vi "Scaled Value.vi"(8 "error in":errorcluster, 11 "Sensor in":refnum<class "Sensor.lvclass">) -> (0 "error out":errorcluster, 2 "Scaled Value":dbl, 3 "Sensor out":refnum<class "Sensor.lvclass">)   [LabVIEW 2026, in "Sensor.lvclass"]
doc: "Returns the sensor's Value multiplied by its Gain. Both fields are read through the class's own Read accessors; the object passes through unchanged."
uses:
  Sensor.lvclass
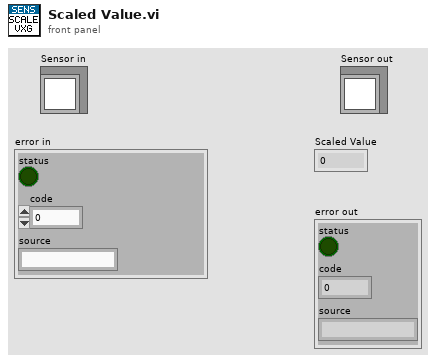
[diagram p1: front panel]
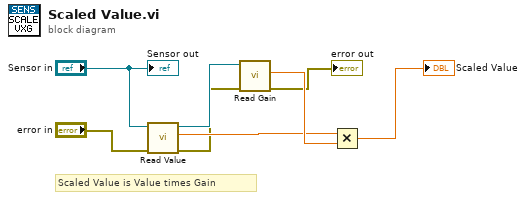
[diagram p0: block diagram]
diagram:
  # "Scaled Value is Value times Gain"
  n1 = call-dynamic "Read Value.vi"("error in (no error)"="error in", "Sensor in"="Sensor in") -> ("error out"=w3:errorcluster, "Value"=w5:dbl, "Sensor out"=w4:refnum<class "Sensor.lvclass">)  [unwired: 7 in]
  n2 = call-dynamic "Read Gain.vi"("error in (no error)"=w3, "Sensor in"=w4) -> ("error out"=→"error out":errorcluster, "Gain"=w7:dbl)  [unwired: 7 in, 1 out]
  n3 = Multiply(x=w5, y=w7) -> (x*y=→"Scaled Value":dbl)
  "Sensor out" <- "Sensor in"
